vi "Read Host Key Data.vi"(8 "error in (no error)":errorcluster, 11 "host key":T1) -> (0 "error out":errorcluster, 2 "host key data":T2)   [LabVIEW 2017, in "libssh2.lvlib"]
doc: "Read the data of a host key."
uses:
  libssh2.lvlib
  libssh2_knownhost.ctl
  Host Key Refnum.ctl
  Acquire Host Key Database.vi
  Release Host Key Database.vi
  Not A Host Key.vi
  <vilib>/Utility/error.llb/Error Cluster From Error Code.vi
  Read Host Key Refnum.vi
  Read Host Key Database Refnum.vi
  <vilib>/Utility/semaphor.llb/Acquire Semaphore.vi
  <vilib>/Utility/semaphor.llb/Release Semaphore.vi
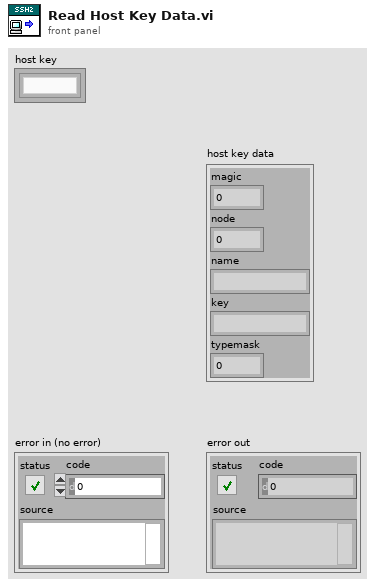
[diagram p1: front panel]
types:
  T1 = typedef "libssh2.lvlib/Host Key Refnum.ctl" = refnum<k1>
  T2 = typedef "libssh2.lvlib/libssh2_knownhost.ctl" = cluster{"magic":u32, "node":u64, "name":string, "key":string, "typemask":i32}
  T3 = cluster{"magic":u32, "node":u64, "name":u64, "key":u64, "typemask":i32}
  T4 = cluster{"magic":u32, "node":u32, "name":u32, "key":u32, "typemask":i32}
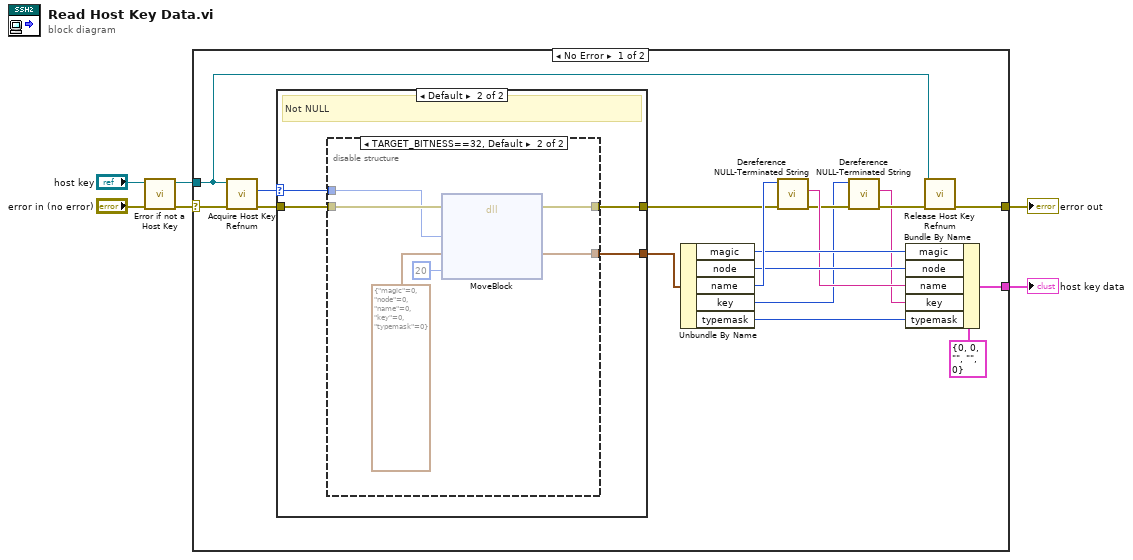
[diagram p0: block diagram]
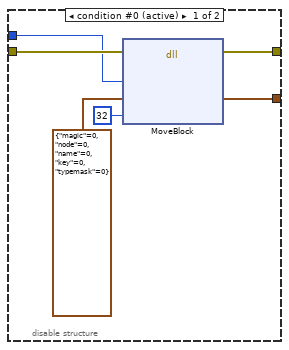
[diagram p3: hidden frame]
diagram:
  n1 = call "Error if not a Host Key.vi"("error in (no error)"="error in (no error)", "host key"="host key") -> ("error out"=w3:errorcluster, "host key out"=w1:T1)  [unwired: 8 in]
  n2 = case shown="No Error" w3 {
    selector: w3 -> [w15 w42]
    tunnel: [w24 _] -> w6
    tunnel: w1 -> [w7 _]
    tunnel: [w8 w42] -> w5
    frame No Error {
      n3 = call "Acquire Host Key Refnum.vi"("error in (no error)"=w15, "host key"=w7) -> ("error out"=w22:errorcluster, "libssh2_knownhost*"=w13:u64)  [unwired: 8 in]
      n4 = case shown="Default" w13 {
        selector: w13 -> [_ w26]
        tunnel: w22 -> [w25 w29]
        tunnel: [_ w28] -> w21
        tunnel: [w25 w27] -> w14
        frame 0 {
          # "NULL"
        }
        frame Default {
          # "Not NULL"
          n5 = disable-structure shown="TARGET_BITNESS==32, Default" {
            disable-tunnel: w29 -> [w35 w41]
            disable-tunnel: [w33 w39] -> w28
            disable-tunnel: [w32 w38] -> w27
            disable-tunnel: w26 -> [w31 w37]
            frame condition #0 (active) {
              n6 = dll-call lib="LabVIEW" fn="MoveBlock"(error in=w35, "ps"=w31, T3 {"magic"=0, "node"=0, "name"=0, "key"=0, "typemask"=0}, "size"=i64 32) -> (error out=w32:errorcluster, w33:T3)  [unwired: 5 in, 1 out]
            }
            frame condition #1 {
              n7 = dll-call lib="LabVIEW" fn="MoveBlock"(error in=w41, "ps"=w37, T4 {"magic"=0, "node"=0, "name"=0, "key"=0, "typemask"=0}, "size"=i64 20) -> (error out=w38:errorcluster, w39:T4)  [unwired: 5 in, 1 out]
            }
          }
        }
      }
      n8 = Unbundle By Name(w21) -> ("magic"=w19:u32, "node"=w18:u64, "name"=w20:u64, "key"=w10:u64, "typemask"=w16:i32)
      n9 = call "Dereference NULL-Terminated String.vi"("error in (no error)"=w14, "char*"=w20) -> ("error out"=w12:errorcluster, "string"=w17:string)  [unwired: 8 in]
      n10 = call "Dereference NULL-Terminated String.vi"("error in (no error)"=w12, "char*"=w10) -> ("error out"=w11:errorcluster, "string"=w9:string)  [unwired: 8 in]
      n11 = Bundle By Name(cluster=T2 {"magic"=0, "node"=0, "name"="", "key"="", "typemask"=0} ("libssh2_knownhost"), "magic"=w19, "node"=w18, "name"=w17, "key"=w9, "typemask"=w16) -> (w24:T2)
      n12 = call "Release Host Key Refnum.vi"("error in (no error)"=w11, "host key"=w7) -> ("error out"=w8:errorcluster)  [unwired: 9 in]
    }
    frame Error {
    }
  }
  "host key data" <- w6
  "error out" <- w5
